vi "VIH ProjFile - Cluster - Write.vi"(8 "error in":errorcluster, 10 "Ctl Refnum":refnum<vi>, 11 "XML Parent Item":refnum<k20>) -> (0 "error out":errorcluster, 3 "dup XML Parent Item":refnum<k20>)   [LabVIEW 2014]
doc: "::: VI Helpeks :::\nCopyright (c) 2000-2026 Konstantin Shifershteyn. All rights reserved."
uses:
  <vilib>/xml/Close Reference(Node).vi
  <resource>/objmgr/DOMUserDefRef.rc
  <vilib>/xml/NI_XML.lvlib
panel:
  # "VI Helpeks\nCopyright (c) 2012-2026 Konstantin Shifershteyn"
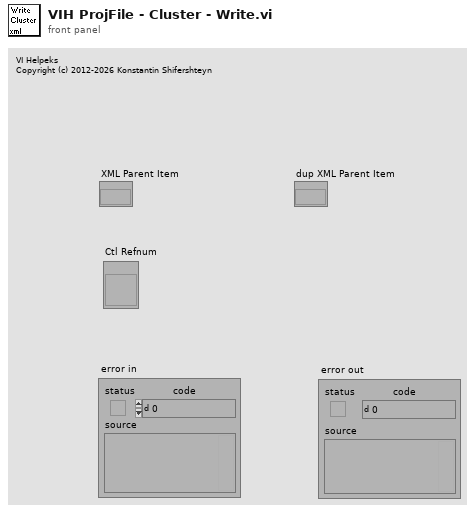
[diagram p1: front panel]
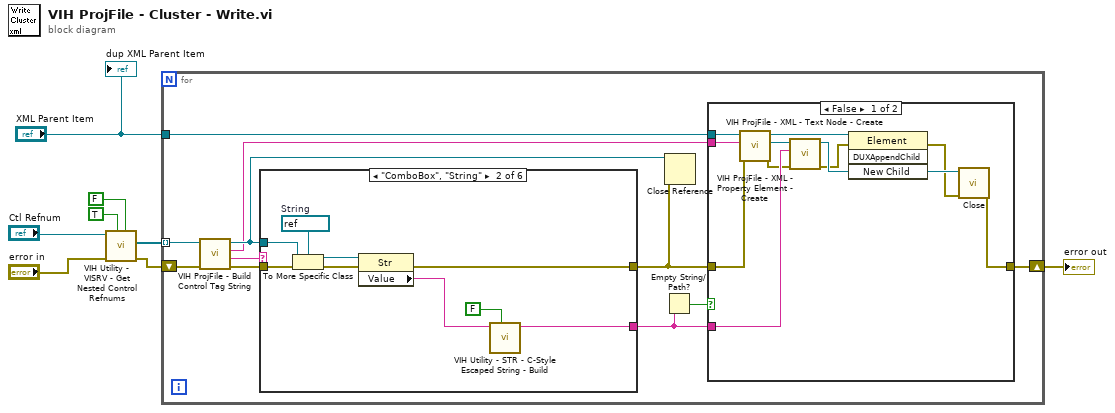
[diagram p0: block diagram]
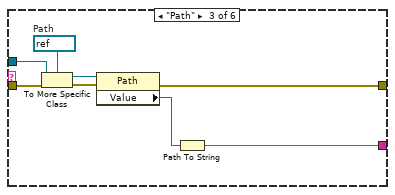
[diagram p4: hidden frame]
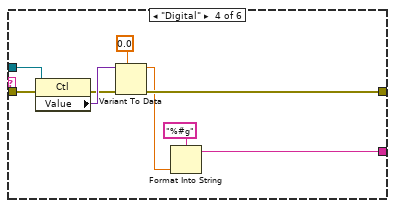
[diagram p5: hidden frame]
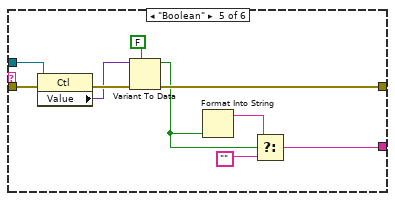
[diagram p6: hidden frame]
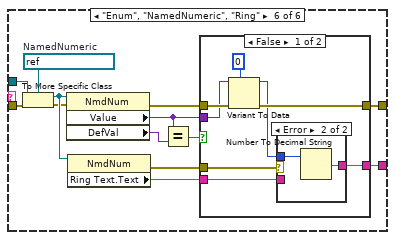
[diagram p7: hidden frame]
diagram:
  n1 = call "VIH Utility - VISRV - Get Nested Control Refnums.vi"("array element (T)"=FALSE, "cluster members (T)"=TRUE, "error in"="error in", "Ctl Refnum"="Ctl Refnum") -> ("error out"=w4:errorcluster, "nested Ctl Refnums"=w5:refnum<vi>[])  [unwired: 5 in, 1 out]
  n2 = for {
    tunnel: w5 -> [w19] mode=indexing
    shift-right: [w10] -> w1
    shift-left: w4 -> [w16]
    tunnel: "XML Parent Item" -> [w13]
    n3 = call "VIH ProjFile - Build Control Tag String.vi"("error in"=w16, "Ctl Refnum"=w19) -> ("error out"=w18:errorcluster, "Control Class"=w17:string, "Control Tag"=w9:string, "dup Ctl Refnum"=w15:refnum<vi>)  [unwired: 5 in, 1 out]
    n4 = case shown="\"ComboBox\", \"String\"" w17 {
      tunnel: w15 -> [_ w40 w44 w50 w64 w75]
      tunnel: w18 -> [w32 w39 w46 w51 w63 w76]
      tunnel: [w32 w41 w48 w55 w66 w80] -> w11
      tunnel: [_ w35 w49 w53 w60 w79] -> w12
      frame Default {
      }
      frame "ComboBox", "String" {
        w36 = refnum<vi> refnum  # String
        n5 = To More Specific Class(target class=w36, reference=w40, error in=w39) -> (specific class reference=w37:refnum<vi>, error out=w38:errorcluster)
        n6 = property class="Str"(reference=w37, error in=w38) -> (error out=w41:errorcluster, "Value"=w34:string)  [unwired: 1 out]
        n7 = call "VIH Utility - STR - C-Style Escaped String - Build.vi"("Escape space char (T)"=FALSE, "String in"=w34) -> ("String out"=w35:string)  [unwired: 9 in]
      }
      frame "Path" {
        w43 = refnum<vi> refnum  # Path
        n8 = To More Specific Class(target class=w43, reference=w44, error in=w46) -> (specific class reference=w42:refnum<vi>, error out=w45:errorcluster)
        n9 = property class="Path"(reference=w42, error in=w45) -> (error out=w48:errorcluster, "Value"=w47:path)  [unwired: 1 out]
        n10 = Path To String(path=w47) -> (string=w49:string)
      }
      frame "Digital" {
        n11 = property class="Ctl"(reference=w50, error in=w51) -> (error out=w56:errorcluster, "Value"=w58:variant)  [unwired: 1 out]
        n12 = Variant To Data(error in=w56, type=0.0, Variant=w58) -> (data=w54:dbl, error out=w55:errorcluster)
        n13 = Format Into String(format string="%#g", w54) -> (resulting string=w53:string)  [unwired: 2 in, 1 out]
      }
      frame "Boolean" {
        n14 = property class="Ctl"(reference=w64, error in=w63) -> (error out=w67:errorcluster, "Value"=w65:variant)  [unwired: 1 out]
        n15 = Variant To Data(error in=w67, type=FALSE, Variant=w65) -> (data=w62:bool, error out=w66:errorcluster)
        n16 = Format Into String(w62) -> (resulting string=w61:string)  [unwired: 3 in, 1 out]
        n17 = Select(t=w61, s=w62, f="") -> (s? t:f=w60:string)
      }
      frame "Enum", "NamedNumeric", "Ring" {
        w74 = refnum<vi> refnum  # NamedNumeric
        n18 = To More Specific Class(target class=w74, reference=w75, error in=w76) -> (specific class reference=w73:refnum<vi>, error out=w72:errorcluster)
        n19 = property class="NmdNum"(reference=w73, error in=w72) -> (error out=w81:errorcluster, "Value"=w71:variant, "DefVal"=w70:variant)  [unwired: 1 out]
        n20 = property class="NmdNum"(reference=w73) -> (error out=w78:errorcluster, "Ring Text.Text"=w77:string)  [unwired: 1 in, 1 out]
        n21 = Equal?(x=w71, y=w70) -> (x = y?=w69:bool)
        n22 = case shown="False" w69 {
          tunnel: w81 -> [w89 w93]
          tunnel: [w88 w93] -> w80
          tunnel: [w86 _] -> w79
          tunnel: w78 -> [w84 _]
          tunnel: w77 -> [w83 _]
          tunnel: w71 -> [w82 _]
          frame False {
            n23 = Variant To Data(error in=w89, type=0, Variant=w82) -> (data=w85:i32, error out=w88:errorcluster)
            n24 = case shown="Error" w84 {
              tunnel: [w90 w92] -> w86
              tunnel: w85 -> [_ w91]
              tunnel: w83 -> [w90 _]
              frame No Error {
              }
              frame Error {
                n25 = Number To Decimal String(number=w91) -> (decimal integer string=w92:string)  [unwired: 1 out]
              }
            }
          }
          frame True {
          }
        }
      }
    }
    n26 = Empty String/Path?(string/path=w12) -> (empty?=w14:bool)
    n27 = Close Reference(reference=w15, error in (no error)=w11) -> ()  [unwired: 1 out]
    n28 = case shown="False" w14 {
      tunnel: w13 -> [w30 _]
      tunnel: w12 -> [w27 _]
      tunnel: w11 -> [w24 w31]
      tunnel: [w20 w31] -> w10
      tunnel: w9 -> [w29 _]
      frame False {
        n29 = call "VIH ProjFile - XML - Property Element - Create.vi"("error in"=w24, "Property Name"=w29, "XML Parent Item"=w30) -> ("error out"=w25:errorcluster, "New Child"=w28:refnum<k20>, "dup XML Parent Item"=w26:refnum<k20>)  [unwired: 6 in]
        n30 = call "VIH ProjFile - XML - Text Node - Create.vi"("error in"=w25, "Data"=w27, "XML Parent Item"=w28) -> ("error out"=w22:errorcluster, "dup XML Parent Item"=w23:refnum<k20>)  [unwired: 7 in]
        n31 = invoke class="Element" method="DUXAppendChild"(reference=w26, error in=w22, "New Child"=w23) -> (error out=w21:errorcluster)  [unwired: 1 in, 3 out]
        n32 = call-poly <vilib>:"Close.vi"("error in (no error)"=w21, "node"=w23) -> ("error out"=w20:errorcluster)  [unwired: 7 in]
      }
      frame True {
      }
    }
  }
  "error out" <- w1
  "dup XML Parent Item" <- "XML Parent Item"
